vi "Sous_VI_acq_ligne.vi"(0 "Seuil":i32=100, 11 "error in (no error)":errorcluster) -> (4 "x > y ?":bool[](array[boolean]), 6 "Décalage":u32(graph), 8 "G/D ?":bool, 10 "4 LED gauches":bool[](array[boolean]), 14 "error out":errorcluster, 15 "4 LED droite":bool[](array[boolean]))   [LabVIEW 2017]
doc: "The myRIO Project template acquires acceleration data from the onboard accelerometer and displays the changes of acceleration values in a waveform chart."
uses:
  <vilib>/myRIO/Instrument Drivers/Onboard IO/I2C/typedefs/I2C User Configuration.ctl
  <vilib>/myRIO/Instrument Drivers/Onboard IO/I2C/typedefs/I2C Transfer Rate.ctl
  <vilib>/myRIO/Instrument Drivers/Onboard IO/I2C/typedefs/I2C Reference.ctl
  <vilib>/myRIO/Common/Instrument Driver Framework/Utilities/typedefs/myRIO Generic Hardware Reference.ctl
  <vilib>/myRIO/Common/Instrument Driver Framework/Utilities/typedefs/Hardware Version Enum.ctl
  <vilib>/myRIO/Common/Instrument Driver Framework/Utilities/typedefs/myRIO v1.0 Reference.ctl
  <vilib>/myRIO/Common/Instrument Driver Framework/Utilities/typedefs/Generic FPGA Reference.ctl
  <vilib>/myRIO/Common/Instrument Driver Framework/myRIO v1.0/I2C/typedefs/I2C Channels Enum.ctl
  <vilib>/myRIO/Instrument Drivers/Onboard IO/I2C/typedefs/I2C Configuration.ctl
  <vilib>/userdefined/High Color/nirio_resource_hc.ctl
  <vilib>/myRIO/Common/Instrument Driver Framework/myRIO v1.0/I2C/vis/myRIO v1.1 Open I2C.vi
  <vilib>/myRIO/Common/Instrument Driver Framework/Utilities/vis/Validate Channels.vi
  <vilib>/myRIO/Common/Instrument Driver Framework/myRIO v1.0/I2C/vis/myRIO v1.0 Reserve I2C.vi
  <vilib>/myRIO/Common/Instrument Driver Framework/myRIO v1.0/I2C/vis/myRIO v1.0 Close I2C.vi
  <vilib>/myRIO/Common/Instrument Driver Framework/myRIO v1.0/I2C/vis/myRIO v1.0 Build MUX Configuration I2C.vi
  <vilib>/myRIO/Common/Instrument Driver Framework/myRIO v1.0/Resource Manager/vis/myRIO v1.0 Reserve Channel List.vi
  <vilib>/myRIO/Common/Instrument Driver Framework/myRIO v1.0/I2C/vis/myRIO v1.0 Unreserve I2C.vi
  <vilib>/myRIO/Common/Instrument Driver Framework/myRIO v1.0/Resource Manager/vis/myRIO v1.0 Create Configuration List.vi
  <vilib>/myRIO/Common/Instrument Driver Framework/myRIO v1.0/Resource Manager/vis/myRIO v1.0 Reserve Channel.vi
  <vilib>/myRIO/Common/Instrument Driver Framework/myRIO v1.0/Resource Manager/vis/myRIO v1.0 Unreserve Channel.vi
  <vilib>/myRIO/Common/Instrument Driver Framework/myRIO v1.0/Resource Manager/vis/myRIO v1.0 Unreserve Channel List.vi
  <vilib>/myRIO/Common/Instrument Driver Framework/myRIO v1.0/Resource Manager/vis/myRIO v1.0 Build Mutex Name.vi
  <vilib>/Utility/VariantDataType/GetNumericInfo.vi
  <vilib>/Utility/error.llb/Error Cluster From Error Code.vi
  <vilib>/myRIO/Common/Instrument Driver Framework/myRIO v1.0/myRIO v1.1 Open.vi
  <vilib>/myRIO/Common/Instrument Driver Framework/Utilities/vis/IO Manager.vi
  <vilib>/myRIO/Common/Instrument Driver Framework/Utilities/vis/Configuration Manager.vi
  <vilib>/myRIO/Common/Instrument Driver Framework/myRIO v1.0/Resource Manager/vis/myRIO v1.0 Configure IO.vi
  <vilib>/myRIO/Common/Instrument Driver Framework/myRIO v1.0/myRIO v1.0 Close.vi
  <vilib>/myRIO/Common/Instrument Driver Framework/myRIO v1.0/I2C/vis/myRIO v1.0 Configure I2C.vi
  <vilib>/myRIO/Common/Instrument Driver Framework/myRIO v1.0/I2C/vis/myRIO v1.0 Read I2C.vi
  <vilib>/myRIO/Common/Instrument Driver Framework/myRIO v1.0/I2C/vis/myRIO v1.0 Shutdown I2C.vi
  <vilib>/myRIO/Instrument Drivers/Onboard IO/I2C/vis/myRIO I2C Open.xnode
  <vilib>/myRIO/Instrument Drivers/Onboard IO/I2C/I2C.lvlib
panel:
  out "tableau décimé":u8[](array[numeric])
  out "Bytes Read":u8[](array[numeric])
  in  "I2C User Configuration":T1
  in  "Channel Name":tag="A/I2C"
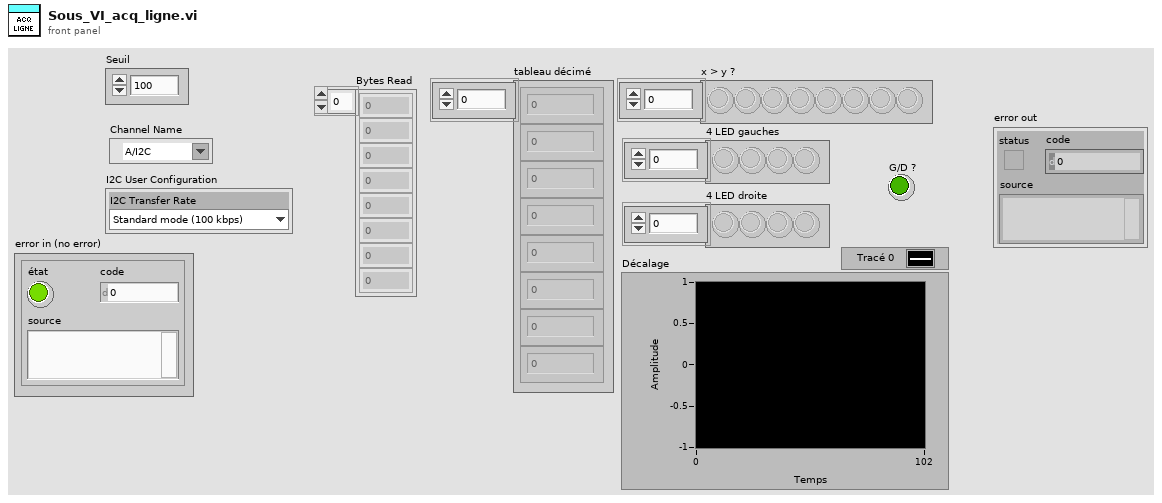
[diagram p1: front panel]
types:
  T1 = typedef "I2C.lvlib/I2C User Configuration.ctl" = cluster{"I2C Transfer Rate":T2}
  T2 = typedef "I2C.lvlib/I2C Transfer Rate.ctl" = enum16{"Standard mode (100 kbps)", "Fast mode (400 kbps)"}
  T3 = typedef "I2C.lvlib/I2C Reference.ctl" = cluster{"myRIO Reference":T4, "I2C Channels Enum":T8, "I2C Configuration":T9}
  T4 = typedef "myRIO Generic Hardware Reference.ctl" = cluster{"myRIO Model":T5, "myRIO Hardware Reference":T6}
  T5 = typedef "Hardware Version Enum.ctl" = enum16{"Unknown", "myRIO-1900", "myRIO-1950", "roboRIO", "NI ELVIS RIO CM"}
  T6 = typedef "myRIO v1.0 Reference.ctl" = cluster{"Generic FPGA Reference":T7, "Allow multiple opens":bool}
  T7 = typedef "Generic FPGA Reference.ctl" = refnum<k20>
  T8 = typedef "I2C Channels Enum.ctl" = enum16{"Not Connected", "A/I2C", "B/I2C", "I2C/I2C"}
  T9 = typedef "I2C.lvlib/I2C Configuration.ctl" = cluster{"I2C Transfer Rate":T2}
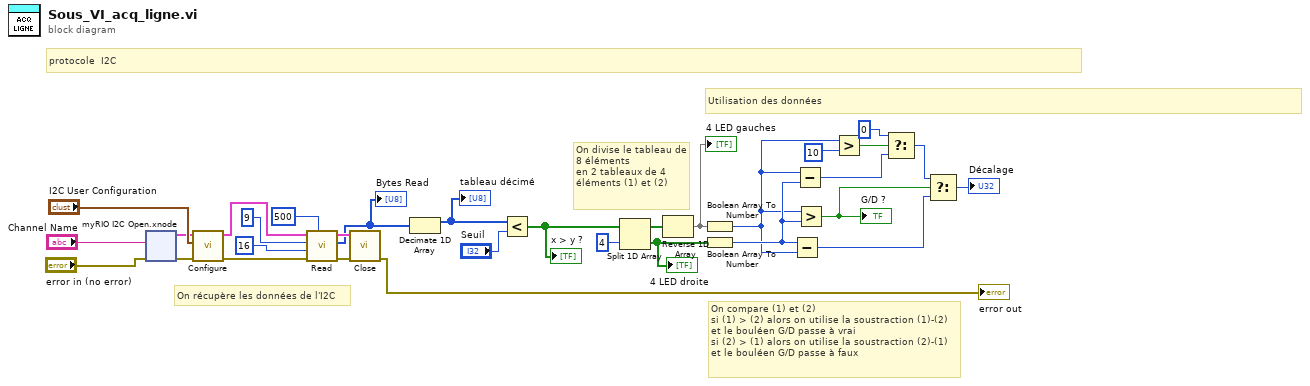
[diagram p0: block diagram]
diagram:
  # "Utilisation des données"
  # "On compare (1) et (2)\nsi (1) > (2) alors on utilise la soustraction (1)-(2)\net le bouléen G/D passe à vrai\nsi (2) > (1) alors on utilise la soustraction (2)-(1)\net le bouléen G/D passe à faux"
  # "On divise le tableau de 8 éléments \nen 2 tableaux de 4 éléments (1) et (2)"
  # "On récupère les données de l'I2C"
  # "protocole  I2C"
  n1 = xnode "myRIO I2C Open.xnode"("error in (no error)"="error in (no error)", "Channel Name"="Channel Name") -> ("error out"=w11:errorcluster, "I2C Ref Out"=w12:T3)  [unwired: 1 in]
  n2 = call <vilib>:"Configure.vi"("error in (no error)"=w11, "I2C User Configuration"="I2C User Configuration", "I2C Ref In"=w12) -> ("error out"=w29:errorcluster, "I2C Ref Out"=w30:T3)  [unwired: 7 in]
  n3 = call <vilib>:"Read.vi"("Timeout ms (1000)"=500, "error in (no error)"=w29, "Byte Count"=u32 16, "Slave Address (7-bit)"=u8 9, "I2C Ref In"=w30) -> ("error out"=w27:errorcluster, "Bytes Read"=w23:u8[], "I2C Ref Out"=w28:T3)  [unwired: 3 in]
  "Bytes Read" <- w23
  n4 = call <vilib>:"Close.vi"("error in (no error)"=w27, "I2C Ref In"=w28) -> ("error out"=→"error out":errorcluster)  [unwired: 9 in]
  n5 = Decimate 1D Array(w23) -> (w22:u8[])  [unwired: 1 out]
  "tableau décimé" <- w22
  n6 = Less?(x=w22, y="Seuil") -> (x < y?=w20:bool[])
  "x > y ?" <- w20
  n7 = Split 1D Array(array=w20, index=4 ("indice")) -> (first subarray=w18:bool[], second subarray=w9:bool[])
  "4 LED droite" <- w9
  n8 = Reverse 1D Array(array=w18) -> (reversed array=w10:bool[])
  "4 LED gauches" <- w10
  n9 = Boolean Array To Number(Boolean array=w10) -> (number=w3:u32)
  n10 = Boolean Array To Number(Boolean array=w9) -> (number=w16:u32)
  n11 = Subtract(x=w16, y=w3) -> (x-y=w15:u32)
  n12 = Subtract(x=w3, y=w16) -> (x-y=w4:u32)
  n13 = Greater?(x=w3, y=w16) -> (0:w17:bool)
  "G/D ?" <- w17
  n14 = Greater?(x=w3, y=u32 10) -> (0:w7:bool)
  n15 = Select(t=u32 0, s=w7, f=w4) -> (s? t:f=w6:u32)
  n16 = Select(t=w6, s=w17, f=w15) -> (s? t:f=→"Décalage":u32)
